vi "Set Channel - Analog Input.vi"(8 "error in (no error)":errorcluster, 9 "ADC Number":T1=-1, 10 "Tag":string, 11 "CTI_GPIO_DigitalOut in":refnum<class "CTI_AnalogIn.lvclass">) -> (0 "error out":errorcluster, 3 "CTI_GPIO_DigitalOut out":refnum<class "CTI_AnalogIn.lvclass">)   [LabVIEW 2021, in "CTI_AnalogIn.lvclass"]
uses:
  CTI_AnalogIn.lvclass
  <vilib>/CTI/CTI Drivers/CTI/ADC Number.ctl
  <vilib>/CTI/CTI Drivers/CTI/CTI.lvlib
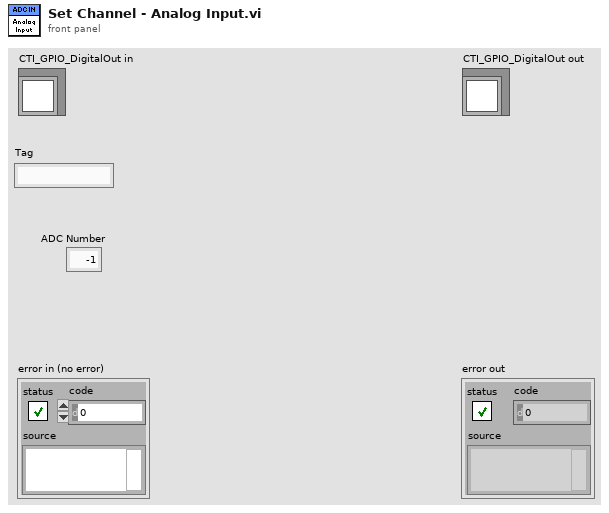
[diagram p1: front panel]
types:
  T1 = typedef "CTI.lvlib/ADC Number.ctl" = i8
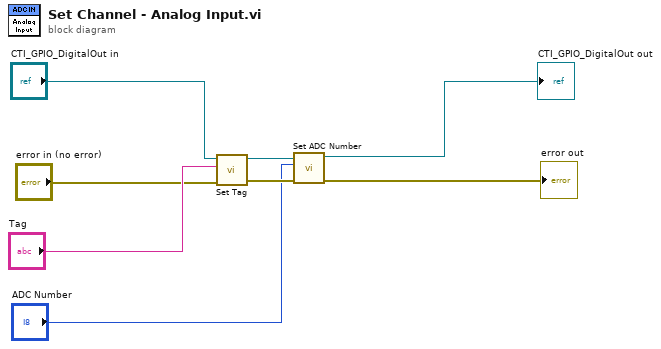
[diagram p0: block diagram]
diagram:
  n1 = call-dynamic "Set Tag.vi"("error in (no error)"="error in (no error)", "Tag"="Tag", "CTI_GPIO_DigitalOut in"="CTI_GPIO_DigitalOut in") -> ("error out"=w4:errorcluster, "CTI_GPIO_DigitalOut out"=w5:refnum<class "CTI_AnalogIn.lvclass">)  [unwired: 7 in]
  n2 = call-dynamic "Set ADC Number.vi"("error in (no error)"=w4, "ADC Number"="ADC Number", "CTI_AnalogIn in"=w5) -> ("error out"=→"error out":errorcluster, "CTI_AnalogIn out"=→"CTI_GPIO_DigitalOut out":refnum<class "CTI_AnalogIn.lvclass">)  [unwired: 7 in]
